vi "CIVI Read Mode Session.vi"(8 "error in":errorcluster, 11 "VISA Session in":refnum<visa-resource-name>="TCPIP0::127.0.0.1::5025::SOCKET") -> (0 "error out":errorcluster, 2 "Mode":string, 3 "VISA Session out":refnum<visa-resource-name>)   [LabVIEW 2026]
doc: "Queries RAD:MODE? through an existing VISA session.\nReturns the response as a mode string.\nDoes not open or close the session."
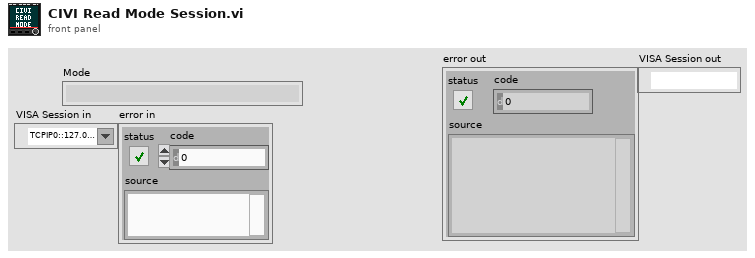
[diagram p1: front panel]
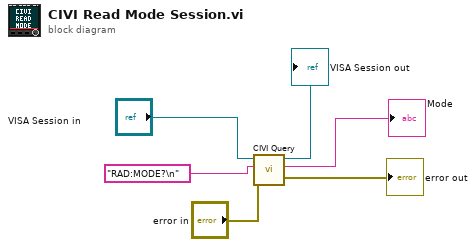
[diagram p0: block diagram]
diagram:
  n1 = call "CIVI Query.vi"("error in"="error in", "write buffer"="RAD:MODE?\n", "VISA Session in"="VISA Session in") -> ("error out"=→"error out":errorcluster, "read buffer"=→"Mode":string, "VISA Session out"=→"VISA Session out":refnum<visa-resource-name>)  [unwired: 6 in]
